vi "Sous_VI_correction.vi"(8 "G/D ?":bool, 11 "Décalage":u32(graph)) -> ()   [LabVIEW 2017]
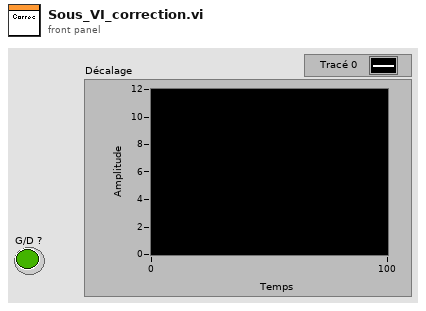
[diagram p1: front panel]
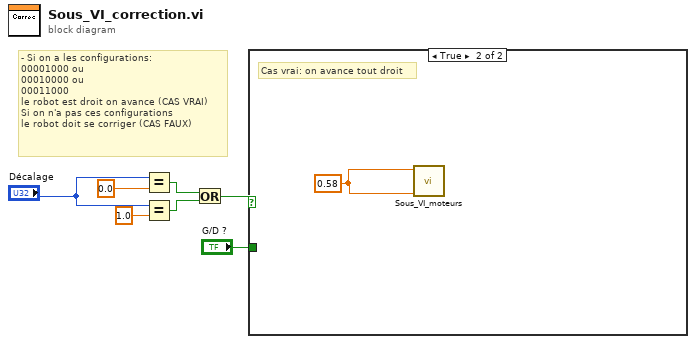
[diagram p0: block diagram]
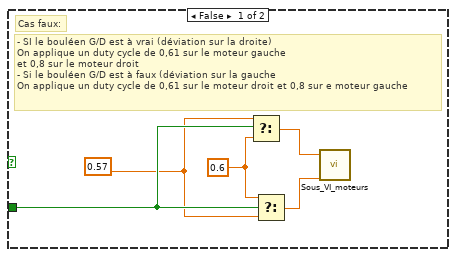
[diagram p2: hidden frame]
diagram:
  # "- Si on a les configurations:\n00001000 ou\n00010000 ou\n00011000\nle robot est droit on avance (CAS VRAI)\nSi on n'a pas ces configurations\nle robot doit se corriger (CAS FAUX)"
  n1 = Equal?(x="Décalage", y=0.0) -> (x = y?=w5:bool)
  n2 = Equal?(x="Décalage", y=1.0) -> (x = y?=w4:bool)
  n3 = Or(x=w5, y=w4) -> (x .or. y?=w3:bool)
  n4 = case shown="True" w3 {
    tunnel: "G/D ?" -> [w9 _]
    frame False {
      w8 = 0.57 ("cas vrai")
      w12 = 0.6 ("cas faux")
      # "Cas faux:"
      # "- SI le bouléen G/D est à vrai (déviation sur la droite)\nOn applique un duty cycle de 0,61 sur le moteur gauche\net 0,8 sur le moteur droit\n- Si le bouléen G/D est à faux (déviation sur la gauche\nOn applique un duty cycle de 0,61 sur le moteur droit et 0,8 sur e moteur gauche"
      n5 = Select(t=w8, s=w9, f=w12) -> (s? t:f=w11:dbl)
      n6 = Select(t=w12, s=w9, f=w8) -> (s? t:f=w10:dbl)
      n7 = call "Sous_VI_moteurs.vi"("Moteur Droit"=w10, "Moteur Gauche"=w11) -> ()  [unwired: 10 in]
    }
    frame True {
      w13 = 0.58
      # "Cas vrai: on avance tout droit"
      n8 = call "Sous_VI_moteurs.vi"("Moteur Droit"=w13, "Moteur Gauche"=w13) -> ()  [unwired: 10 in]
    }
  }
